vi "FuncVI_Sub - Script - Pass single parameter.vi"(5 "Dst VC Handle":T2, 6 "action":enum32{"import", "export"}(ring), 7 "Src VC Handle":T2, 8 "error in":errorcluster, 9 "CE InstanceRef":T1, 10 "Dst var name":string, 11 "Src var name":string) -> (0 "error out":errorcluster)   [LabVIEW 2021]
doc: "::: CalcExpress Toolkit :::\nCopyright (c) 2000-2026 Konstantin Shifershteyn. All rights reserved."
uses:
  cetypes.llb/VarMan Variable Context Handle.ctl
  cetypes.llb/CalcExpress Instance RefNum.ctl
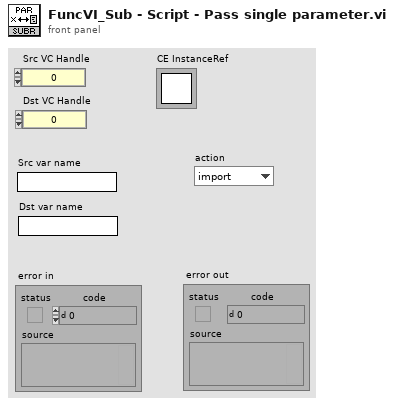
[diagram p1: front panel]
types:
  T1 = typedef "CalcExpress Instance RefNum.ctl" = refnum<k1>
  T2 = typedef "VarMan Variable Context Handle.ctl" = i32
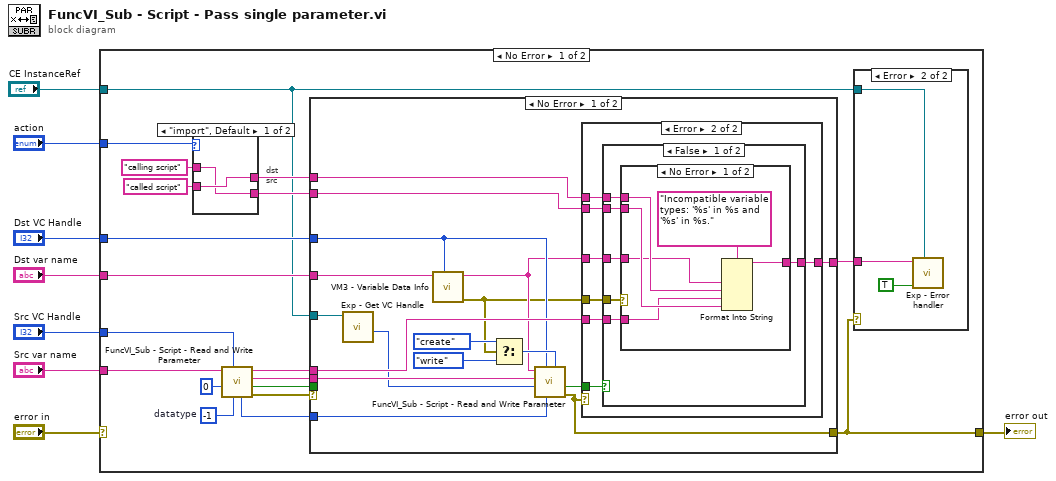
[diagram p0: block diagram]
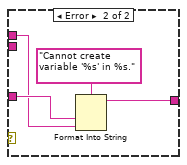
[diagram p5: hidden frame]
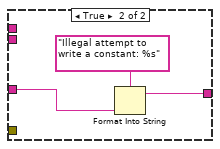
[diagram p6: hidden frame]
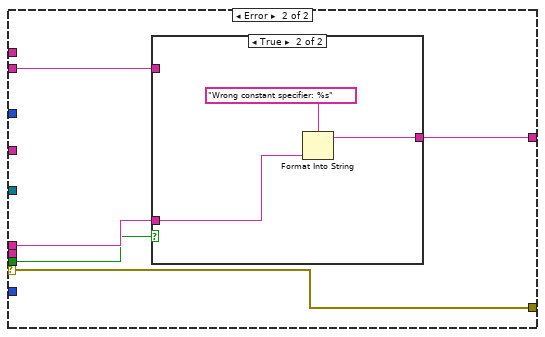
[diagram p7: hidden frame]
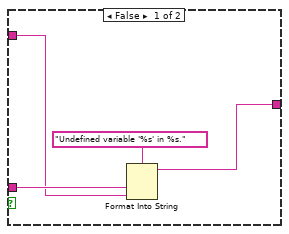
[diagram p8: hidden frame]
diagram:
  n1 = case shown="No Error" "error in" {
    selector: "error in" -> [_ w90]
    tunnel: [w18 w90] -> w7
    tunnel: "Dst var name" -> [w15 _]
    tunnel: "Src var name" -> [w14 _]
    tunnel: "Dst VC Handle" -> [w13 _]
    tunnel: "Src VC Handle" -> [w12 _]
    tunnel: "action" -> [w11 _]
    tunnel: "CE InstanceRef" -> [w10 _]
    frame No Error {
      w17 = -1  # datatype
      # "dst\nsrc"
      n2 = case shown="\"import\", Default" w11 {
        tunnel: [w32 w34] -> w21
        tunnel: "calling script" -> [w31 w34]
        tunnel: [w31 w33] -> w20
        tunnel: "called script" -> [w32 w33]
        frame "import", Default {
        }
        frame "export" {
        }
      }
      n3 = call "FuncVI_Sub - Script - Read and Write Parameter.vi"("var type"=w17, "VC Handle"=w12, "writer ID"=u32 0, "var name/const"=w14) -> ("error out"=w27:errorcluster, "constant?"=w16:bool, "flattened value out"=w26:string, "dup var name/const"=w24:string, "var type out"=w25:u32)  [unwired: 3 in]
      n4 = case shown="No Error" w27 {
        selector: w27 -> [_ w82]
        tunnel: w15 -> [w36 _]
        tunnel: w13 -> [w38 _]
        tunnel: w26 -> [w51 _]
        tunnel: w25 -> [w50 _]
        tunnel: w24 -> [w45 w81]
        tunnel: [w49 w82] -> w18
        tunnel: [w47 w80] -> w19
        tunnel: w21 -> [w46 _]
        tunnel: w20 -> [w48 w79]
        tunnel: w16 -> [_ w78]
        tunnel: w10 -> [w40 _]
        frame No Error {
          n5 = call "Exp - Get VC Handle.vi"("InstanceRef"=w40) -> ("writer ID"=w39:u32)  [unwired: 5 in, 3 out]
          n6 = call "VM3 - Variable Data Info.vi"("VC Handle"=w38, "name_spec"=w36) -> ("error out"=w35:errorcluster, "dup name_spec"=w37:string)  [unwired: 4 in, 4 out]
          n7 = Select(t=enum16{"create", "destroy", "write", "read"}."create" ("cmd (read)"), s=w35, f=enum16{"create", "destroy", "write", "read"}."write") -> (s? t:f=w41:enum16{"create", "destroy", "write", "read"})
          n8 = call "FuncVI_Sub - Script - Read and Write Parameter.vi"("cmd (read)"=w41, "var type"=w50, "VC Handle"=w38, "writer ID"=w39, "flattened value"=w51, "var name/const"=w37) -> ("error out"=w49:errorcluster, "constant?"=w44:bool)  [unwired: 1 in, 3 out]
          n9 = case shown="Error" w49 {
            tunnel: w35 -> [_ w58]
            tunnel: w37 -> [_ w57]
            tunnel: w48 -> [_ w56]
            tunnel: [_ w55] -> w47
            tunnel: w46 -> [_ w54]
            tunnel: w45 -> [_ w53]
            tunnel: w44 -> [_ w52]
            frame No Error {
            }
            frame Error {
              n10 = case shown="False" w52 {
                tunnel: w58 -> [w64 _]
                tunnel: w57 -> [w63 w75]
                tunnel: w56 -> [w62 _]
                tunnel: [w61 w76] -> w55
                tunnel: w54 -> [w60 _]
                tunnel: w53 -> [w59 _]
                frame False {
                  n11 = case shown="No Error" w64 {
                    tunnel: w63 -> [w66 w74]
                    tunnel: w62 -> [w67 _]
                    tunnel: [w70 w73] -> w61
                    tunnel: w60 -> [w68 w71]
                    tunnel: w59 -> [w65 _]
                    frame No Error {
                      n12 = Format Into String(format string="Incompatible variable types: '%s' in %s and '%s' in %s.", w66, w68, w65, w67) -> (resulting string=w70:string)  [unwired: 2 in, 1 out]
                    }
                    frame Error {
                      n13 = Format Into String(format string="Cannot create variable '%s' in %s.", w74, w71) -> (resulting string=w73:string)  [unwired: 2 in, 1 out]
                    }
                  }
                }
                frame True {
                  n14 = Format Into String(format string="Illegal attempt to write a constant: %s", w75) -> (resulting string=w76:string)  [unwired: 2 in, 1 out]
                }
              }
            }
          }
        }
        frame Error {
          n15 = case shown="True" w78 {
            tunnel: w81 -> [w86 w87]
            tunnel: [w84 w88] -> w80
            tunnel: w79 -> [w83 _]
            frame False {
              n16 = Format Into String(format string="Undefined variable '%s' in %s.", w86, w83) -> (resulting string=w84:string)  [unwired: 2 in, 1 out]
            }
            frame True {
              n17 = Format Into String(format string="Wrong constant specifier: %s", w87) -> (resulting string=w88:string)  [unwired: 2 in, 1 out]
            }
          }
        }
      }
      n18 = case shown="Error" w18 {
        tunnel: w19 -> [_ w30]
        tunnel: w10 -> [_ w28]
        frame No Error {
        }
        frame Error {
          n19 = call "Exp - Error handler.vi"("InstanceRef"=w28, "error in"=TRUE, "error message in"=w30) -> ()  [unwired: 6 in, 3 out]
        }
      }
    }
    frame Error {
    }
  }
  "error out" <- w7
